vi "apply key value pairs.vi"(8 "error in":errorcluster, 9 "values":string[](array[string]), 10 "keys":string[](array[string]), 11 "fixed channel runtime in":refnum<class "MotionModule runtime.lvclass">) -> (0 "error out":errorcluster, 3 "fixed channel runtime out":refnum<class "MotionModule runtime.lvclass">)   [LabVIEW 2017, in "MotionModule runtime.lvclass"]
uses:
  MotionModule runtime.lvclass
  MotionModule runtime.lvclass/MotionModule runtime.ctl
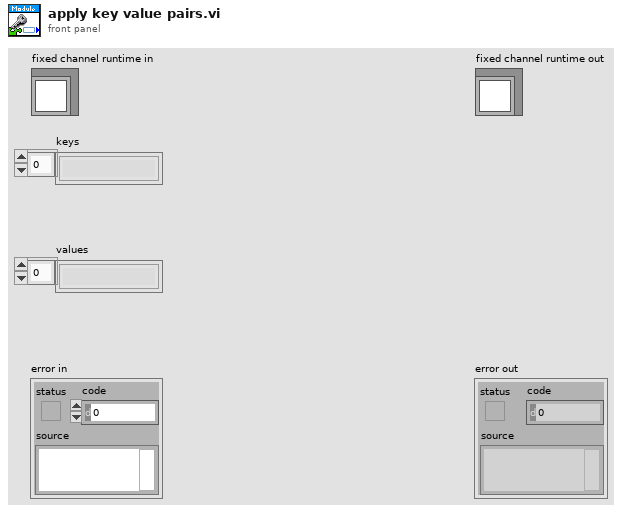
[diagram p1: front panel]
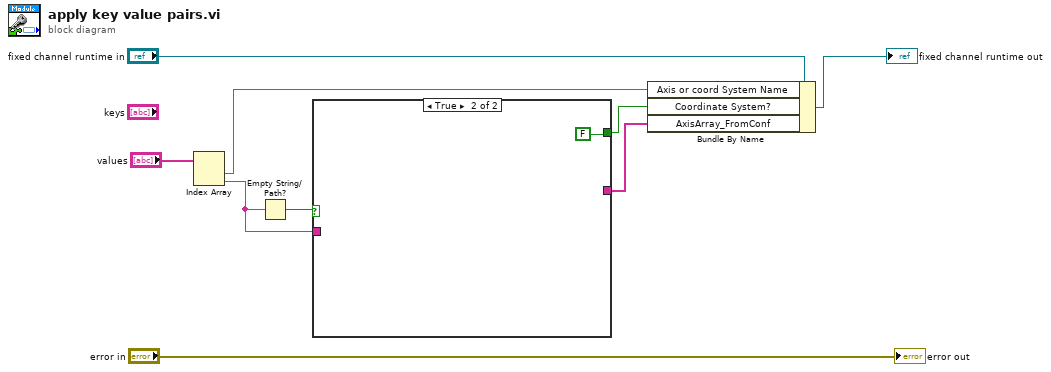
[diagram p0: block diagram]
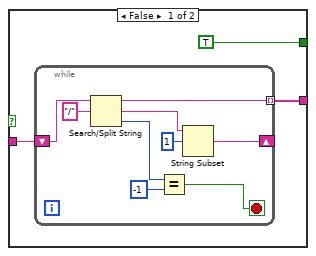
[diagram p2: hidden frame]
diagram:
  n1 = Index Array(array="values") -> (element #1=w5:string, element #2=w2:string)  [unwired: 2 in]
  n2 = Empty String/Path?(string/path=w2) -> (empty?=w3:bool)
  n3 = case shown="True" w3 {
    tunnel: w2 -> [w12 _]
    tunnel: [w11 _] -> w4
    tunnel: [TRUE FALSE] -> w1
    frame False {
      n4 = while {
        tunnel: [w20] -> w11 mode=indexing
        shift-right: [w17] -> _
        shift-left: w12 -> [w16]
        stop <- w13 stop-if-true
        n5 = Search/Split String(string=w16, search string/char (-)="/") -> (substring before match=w20:string, match + rest of string=w19:string, offset of match=w15:i32)  [unwired: 1 in]
        n6 = Equal?(x=w15, y=-1) -> (x = y?=w13:bool)
        n7 = String Subset(string=w19, offset (0)=1) -> (substring=w17:string)  [unwired: 1 in]
      }
    }
    frame True {
    }
  }
  n8 = Bundle By Name(cluster="fixed channel runtime in", "Axis or coord System Name"=w5, "Coordinate System?"=w1, "AxisArray_FromConf"=w4) -> (→"fixed channel runtime out":refnum<class "MotionModule runtime.lvclass">)
  "error out" <- "error in"
